vi "Scale_Graph_Y (SubVI).vi"(6 "AktYSkl":u8, 8 "Divisor":dbl, 9 "Array":dbl[](array[numeric]), 10 "Faktor":dbl, 11 "XYGraph (Eingang)":refnum<vi>) -> ()   [LabVIEW 2014]
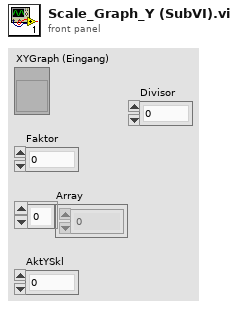
[diagram p1: front panel]
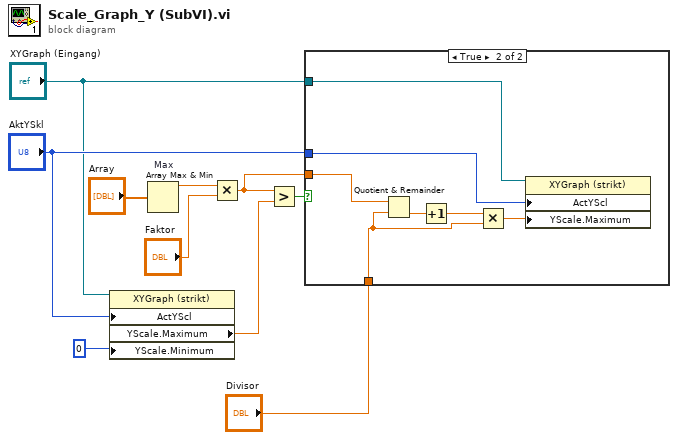
[diagram p0: block diagram]
diagram:
  n1 = property on="Eigenschaftsknoten" class="XYGraph (strikt)"(reference="XYGraph (Eingang)", "ActYScl"="AktYSkl", "YScale.Minimum"=0) -> ("YScale.Maximum"=w7:dbl)  [unwired: 1 in, 2 out]
  n2 = Array Max & Min "Max"(array="Array") -> (max value=w8:dbl)  [unwired: 3 out]
  n3 = Multiply(x=w8, y="Faktor") -> (x*y=w5:dbl)
  n4 = Greater?(x=w5, y=w7) -> (0:w6:bool)
  n5 = case shown="True" w6 {
    tunnel: w5 -> [_ w15]
    tunnel: "AktYSkl" -> [_ w13]
    tunnel: "XYGraph (Eingang)" -> [_ w12]
    tunnel: "Divisor" -> [_ w11]
    frame False {
    }
    frame True {
      n6 = Quotient & Remainder(x=w15, y=w11) -> (floor(x/y)=w16:dbl)  [unwired: 1 out]
      n7 = Increment(x=w16) -> (x+1=w17:dbl)
      n8 = Multiply(x=w17, y=w11) -> (x*y=w14:dbl)
      n9 = property on="Eigenschaftsknoten" class="XYGraph (strikt)"(reference=w12, "ActYScl"=w13, "YScale.Maximum"=w14) -> ()  [unwired: 1 in, 2 out]
    }
  }
